vi "set Detector Mode.vi"(6 "Detect Auto?":bool, 8 "error in (no error)":errorcluster, 9 "Trace Index":u32=1 min=1, 10 "Detector Type":T1=enum."Auto Peak", 11 "Keysight 9020A in":refnum<class "Keysight 9020A.lvclass">) -> (0 "error out":errorcluster, 3 "Keysight 9020A out":refnum<class "Keysight 9020A.lvclass">)   [LabVIEW 2023, in "Spectrum Analyzer.lvlib" / "Keysight 9020A.lvclass"]
uses:
  Keysight 9020A.lvclass
  TYPE DEFINITION/TYPE Detect Mode Select.ctl
  Keysight 9020A.lvclass/Keysight 9020A.ctl
  Spectrum Analyzer.lvlib
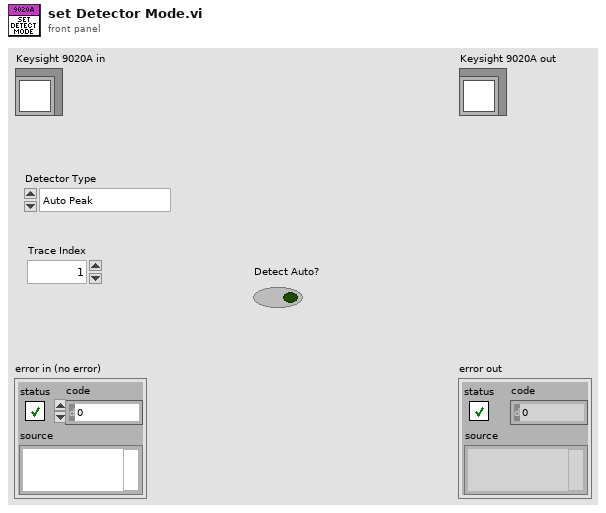
[diagram p1: front panel]
types:
  T1 = typedef "Spectrum Analyzer.lvlib/TYPE Detect Mode Select.ctl" = enum16{"Det Auto (Normal)", "Auto Peak", "Positive Peak", "Negative Peak", "Sample", "RMS", "Average", "Quasipeak", "CISPR Average", "RMS Average"}
  T2 = typedef "Spectrum Analyzer.lvlib/TYPE Measurement Preset.ctl" = enum16{"Sweep SA Mode", "Channel Power", "Occupied BW", "ACP", "Spurious Emission", "Spurious Emission Mask", "Burst Power (Transmit Power)"}
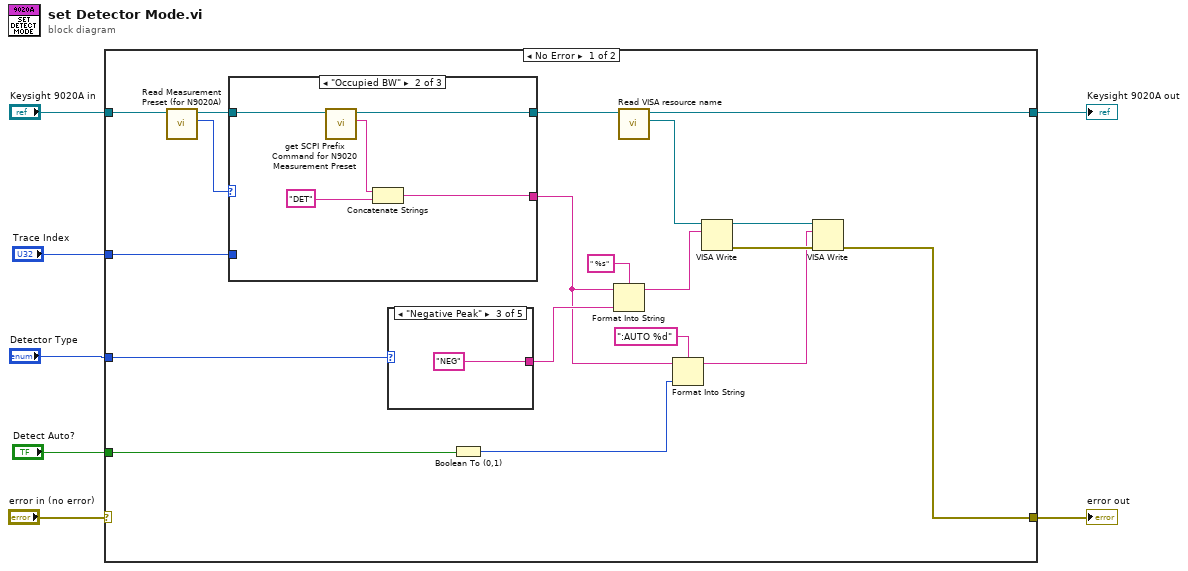
[diagram p0: block diagram]
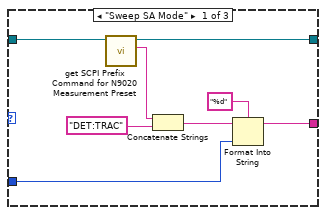
[diagram p2: hidden frame]
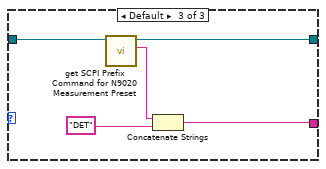
[diagram p3: hidden frame]
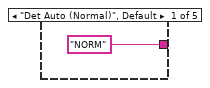
[diagram p4: hidden frame]
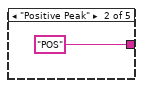
[diagram p5: hidden frame]
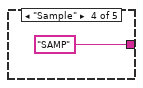
[diagram p6: hidden frame]
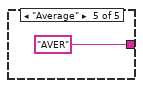
[diagram p7: hidden frame]
diagram:
  n1 = case shown="No Error" "error in (no error)" {
    selector: "error in (no error)" -> [_ w50]
    tunnel: "Keysight 9020A in" -> [w18 w51]
    tunnel: [w21 w51] -> w6
    tunnel: [w24 w50] -> w4
    tunnel: "Detector Type" -> [w26 _]
    tunnel: "Trace Index" -> [w15 _]
    tunnel: "Detect Auto?" -> [w25 _]
    frame No Error {
      n2 = call "Read Measurement Preset (for N9020A).vi"("Keysight 9020A in"=w18) -> ("Measurement Preset"=w16:T2, "Keysight 9020A out"=w17:refnum<class "Keysight 9020A.lvclass">)  [unwired: 8 in, 1 out]
      n3 = case shown="\"Occupied BW\"" w16 {
        tunnel: [w33 w38 w43] -> w22
        tunnel: w17 -> [w31 w36 w41]
        tunnel: w15 -> [w28 _ _]
        tunnel: [w27 w35 w40] -> w11
        frame "Sweep SA Mode" {
          n4 = call "get SCPI Prefix Command for N9020 Measurement Preset.vi"("Keysight 9020A in"=w31) -> ("SCPI Prefix Command"=w32:string, "Keysight 9020A out"=w33:refnum<class "Keysight 9020A.lvclass">)  [unwired: 8 in, 1 out]
          n5 = Concatenate Strings(w32, "DET:TRAC") -> (w29:string)
          n6 = Format Into String(format string="%d", initial string=w29, w28) -> (resulting string=w27:string)  [unwired: 1 in, 1 out]
        }
        frame "Occupied BW" {
          n7 = call "get SCPI Prefix Command for N9020 Measurement Preset.vi"("Keysight 9020A in"=w36) -> ("SCPI Prefix Command"=w37:string, "Keysight 9020A out"=w38:refnum<class "Keysight 9020A.lvclass">)  [unwired: 8 in, 1 out]
          n8 = Concatenate Strings(w37, "DET") -> (w35:string)
        }
        frame Default {
          n9 = call "get SCPI Prefix Command for N9020 Measurement Preset.vi"("Keysight 9020A in"=w41) -> ("SCPI Prefix Command"=w42:string, "Keysight 9020A out"=w43:refnum<class "Keysight 9020A.lvclass">)  [unwired: 8 in, 1 out]
          n10 = Concatenate Strings(w42, "DET") -> (w40:string)
        }
      }
      n11 = case shown="\"Negative Peak\"" w26 {
        tunnel: ["NORM" "POS" "NEG" "SAMP" "AVER"] -> w13
        frame "Det Auto (Normal)", Default {
        }
        frame "Positive Peak" {
        }
        frame "Negative Peak" {
        }
        frame "Sample" {
        }
        frame "Average" {
        }
      }
      n12 = Boolean To (0,1)(Boolean=w25) -> (0, 1=w9:i16)
      n13 = Format Into String(format string=" %s", initial string=w11, w13) -> (resulting string=w12:string)  [unwired: 1 in, 1 out]
      n14 = call "Read VISA resource name.vi"("Keysight 9020A in"=w22) -> ("VISA resource name"=w23:refnum<visa-resource-name>, "Keysight 9020A out"=w21:refnum<class "Keysight 9020A.lvclass">)  [unwired: 8 in, 1 out]
      n15 = Format Into String(format string=":AUTO %d", initial string=w11, w9) -> (resulting string=w8:string)  [unwired: 1 in, 1 out]
      n16 = VISA Write(VISA resource name=w23, write buffer=w12) -> (VISA resource name out=w20:refnum<visa-resource-name>, error out=w19:errorcluster)  [unwired: 1 in, 1 out]
      n17 = VISA Write(VISA resource name=w20, write buffer=w8, error in (no error)=w19) -> (error out=w24:errorcluster)  [unwired: 2 out]
    }
    frame Error {
    }
  }
  "error out" <- w4
  "Keysight 9020A out" <- w6
